vi "Read Multipage ImageJ TIFF Stack.vi"(0 "ImageJ Tif Path":path, 11 "Error In":errorcluster) -> (4 "U8 Stack":u8[][][](array[numeric]), 6 "U8 Image?":bool, 8 "U16 Stack":u16[][][](array[numeric]), 13 "Image Info":T1, 15 "Error Out":errorcluster)   [LabVIEW 2016]
uses:
  ImageJ TIF Type Defs/TIF Read Image Information.ctl
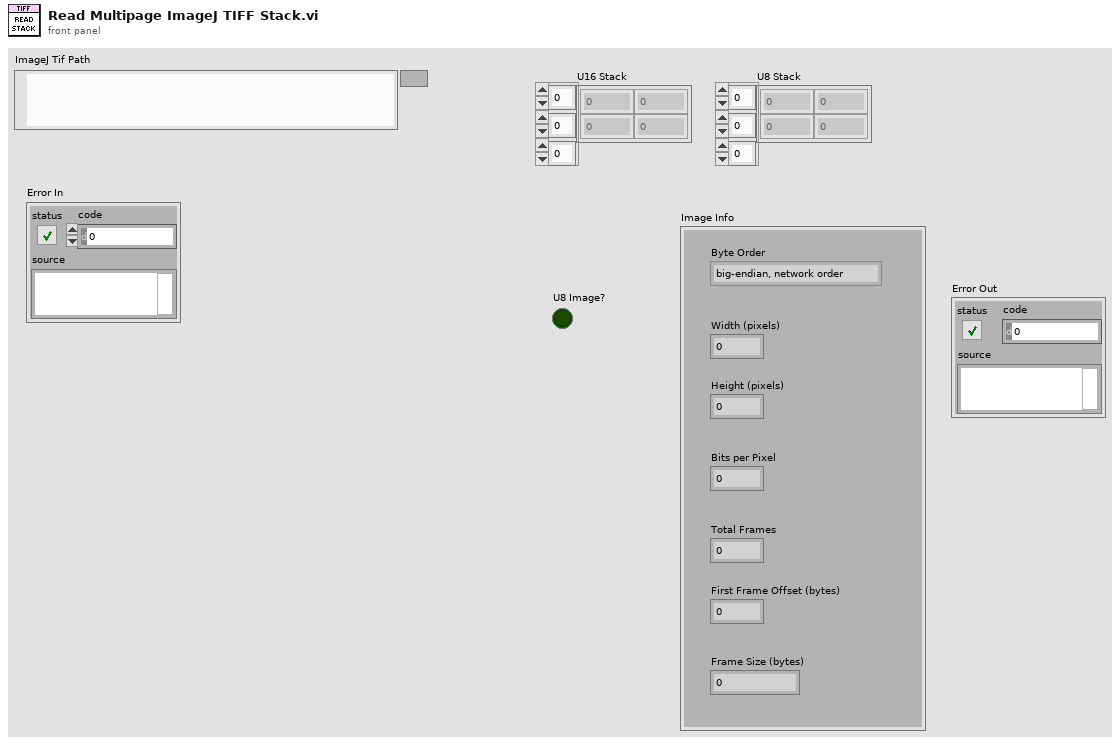
[diagram p1: front panel]
types:
  T1 = typedef "TIF Read Image Information.ctl" = cluster{"Byte Order":enum16{"big-endian, network order", "native, host order", "little-endian"}, "Width (pixels)":i32, "Height (pixels)":i32, "Bits per Pixel":u8, "Total Frames":u32, "First Frame Offset (bytes)":u32, "Frame Size (bytes)":u32}
  T2 = enum16{"big-endian, network order", "native, host order", "little-endian"}
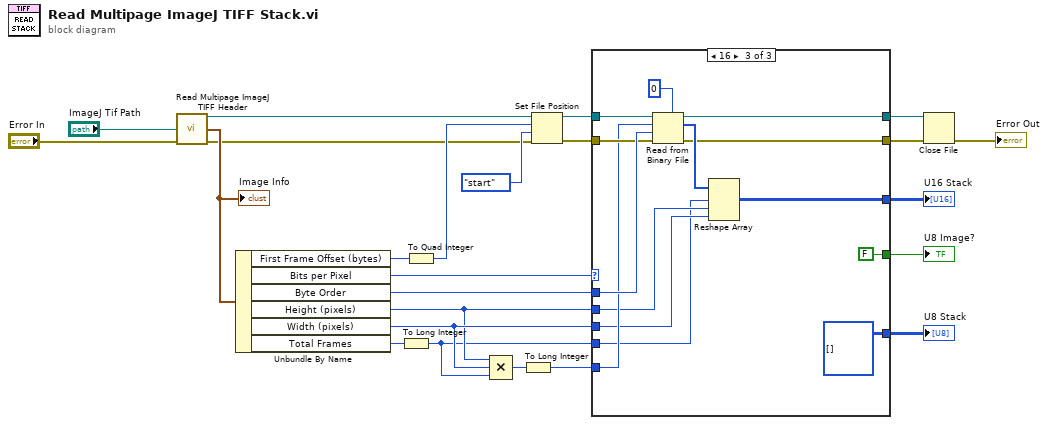
[diagram p0: block diagram]
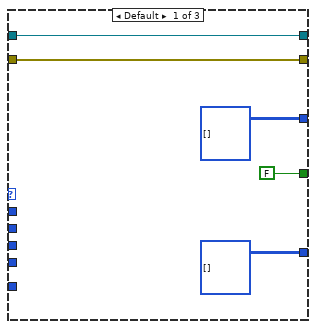
[diagram p2: hidden frame]
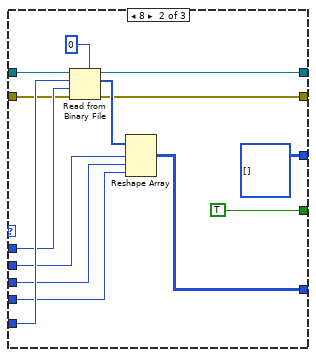
[diagram p3: hidden frame]
diagram:
  n1 = call "Read Multipage ImageJ TIFF Header.vi"("TIFF Path"="ImageJ Tif Path", "Error"="Error In") -> ("TIF Ref"=w22:refnum<file>, "Image Info"=w23:T1, "Error"=w15:errorcluster)  [unwired: 11 in]
  "Image Info" <- w23
  n2 = Unbundle By Name(w23) -> ("First Frame Offset (bytes)"=w20:u32, "Bits per Pixel"=w17:u8, "Byte Order"=w8:T2, "Height (pixels)"=w5:i32, "Width (pixels)"=w6:i32, "Total Frames"=w7:u32)
  n3 = To Long Integer(number=w7) -> (32bit integer=w4:i32)
  n4 = To Quad Integer(1:w20) -> (0:w19:i64)
  n5 = Compound Arithmetic op=MULTIPLY(w5, w6, w4) -> (w3:i32)
  n6 = To Long Integer(number=w3) -> (32bit integer=w14:i32)
  n7 = Set File Position(offset (in bytes) (0)=w19, refnum=w22, from (0:start)=enum16{"start", "end", "current"}."start", error in=w15) -> (refnum out=w18:refnum<file>, error out=w16:errorcluster)
  n8 = case shown="16" w17 {
    tunnel: w18 -> [w29 w43 w57]
    tunnel: w14 -> [_ w41 w47]
    tunnel: w8 -> [_ w40 w55]
    tunnel: w16 -> [w28 w39 w54]
    tunnel: w5 -> [_ w37 w45]
    tunnel: w6 -> [_ w36 w46]
    tunnel: [w29 w35 w52] -> w13
    tunnel: [w28 w34 w51] -> w12
    tunnel: [FALSE TRUE FALSE] -> w11
    tunnel: w4 -> [_ w32 w44]
    tunnel: [u16[][][] [] u16[][][] [] w49] -> w10
    tunnel: [u8[][][] [] w31 u8[][][] []] -> w9
    frame Default {
    }
    frame 8 {
      n9 = Read from Binary File(5:u8 0, 8:w39, 9:w40, 10:w41, 11:w43) -> (0:w34:errorcluster, 2:w38:u8[], 3:w35:refnum<file>)  [unwired: 1 in, 1 out]
      n10 = Reshape Array(w38, w37, w36, w32) -> (w31:u8[][][])
    }
    frame 16 {
      n11 = Read from Binary File(5:u16 0, 8:w54, 9:w55, 10:w47, 11:w57) -> (0:w51:errorcluster, 2:w53:u16[], 3:w52:refnum<file>)  [unwired: 1 in, 1 out]
      n12 = Reshape Array(w53, w44, w45, w46) -> (w49:u16[][][])
    }
  }
  "U8 Image?" <- w11
  "U16 Stack" <- w10
  "U8 Stack" <- w9
  n13 = Close File(refnum=w13, error in=w12) -> (error out=→"Error Out":errorcluster)  [unwired: 1 out]
